vi "DAC Configure.vi"(8 "error in":errorcluster, 11 "DAC HMP4040 in":refnum<class "DAC HMP4040.lvclass">) -> (0 "error out":errorcluster, 3 "DAC HMP4040 out":refnum<class "DAC HMP4040.lvclass">)   [LabVIEW 2019, in "DAC.lvlib" / "DAC HMP4040.lvclass"]
uses:
  DAC HMP4040.lvclass
  C:/Users/krio/Documents/LV_Projects/test-stand/App/DAC/DAC.lvclass
  DAC.lvclass/DAC.ctl
  DAC HMP4040.lvclass/DAC HMP4040.ctl
  <vilib>/Instr/_visa.llb/VISA Configure Serial Port (Instr).vi
  <vilib>/Utility/error.llb/Error Cluster From Error Code.vi
  <vilib>/ErrorRing/Error Ring.xnode
  DAC.lvclass
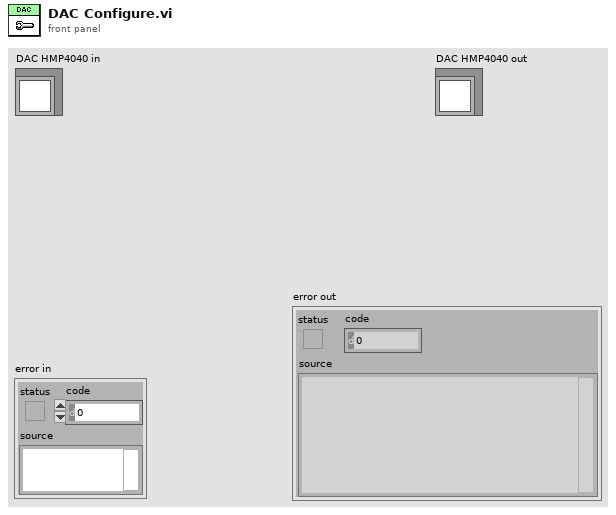
[diagram p1: front panel]
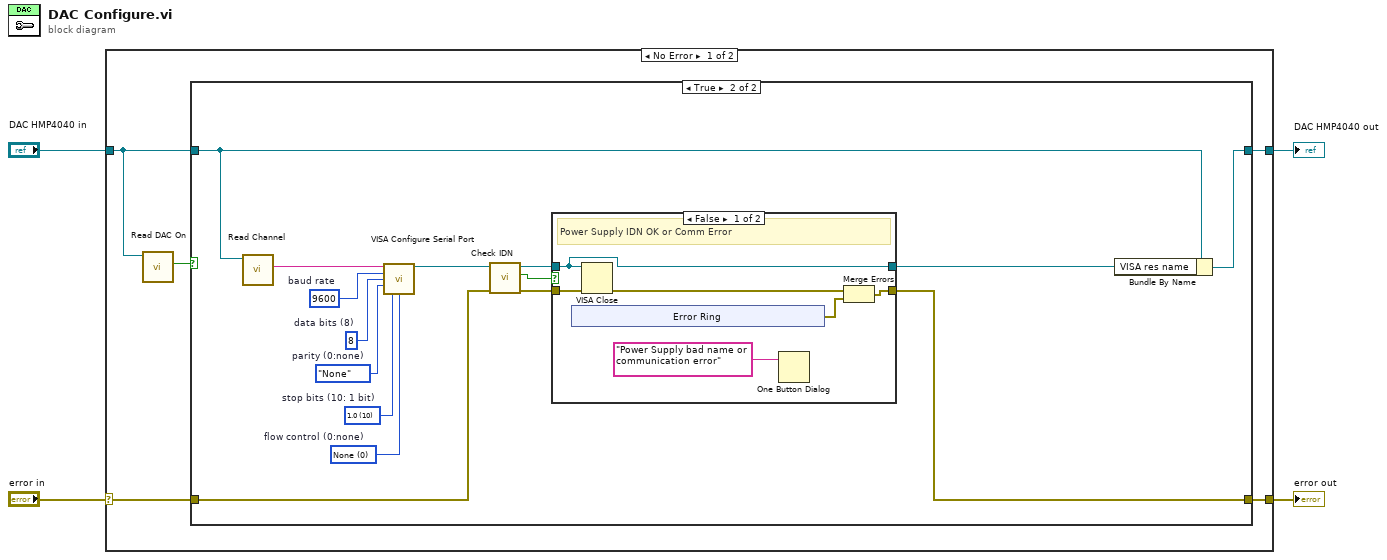
[diagram p0: block diagram]
diagram:
  n1 = case shown="No Error" "error in" {
    selector: "error in" -> [w6 w40]
    tunnel: [w5 w40] -> w4
    tunnel: [w7 w39] -> w3
    tunnel: "DAC HMP4040 in" -> [w9 w39]
    frame No Error {
      n2 = call "Read DAC On.vi"("DAC in"=w9) -> ("DAC On"=w8:bool)  [unwired: 8 in, 2 out]
      n3 = case shown="True" w8 {
        tunnel: w9 -> [w11 w21]
        tunnel: [w11 w26] -> w7
        tunnel: w6 -> [w10 w17]
        tunnel: [w10 w12] -> w5
        frame False {
        }
        frame True {
          w19 = u16 0 items=["None", "XON/XOFF", "RTS/CTS", "XON/XOFF & RTS/CTS", "DTR/DSR", "XON/XOFF & DTR/DSR"]  # flow control (0:none)
          w22 = u16 10 items=["1.0"=10, "1.5"=15, "2.0"=20]  # stop bits (10: 1 bit)
          w23 = enum16{"None", "Odd", "Even", "Mark", "Space"}."None"  # parity (0:none)
          w24 = u16 8  # data bits (8)
          w25 = u32 9600  # baud rate
          n4 = call "Read Channel.vi"("DAC in"=w21) -> ("Channel"=w20:string)  [unwired: 8 in, 2 out]
          n5 = call-poly "VISA Configure Serial Port"("VISA resource name"=w20, "baud rate (9600)"=w25, "data bits (8)"=w24, "parity (0:none)"=w23, "stop bits (10: 1 bit)"=w22, "flow control (0:none)"=w19) -> ("VISA resource name out"=w18:refnum<visa-resource-name>)  [unwired: 8 in, 1 out]
          n6 = call "Check IDN.vi"("error in"=w17, "VISA Refnum in"=w18) -> ("error out"=w13:errorcluster, "IDN OK?"=w14:bool, "VISA Refnum out"=w16:refnum<visa-resource-name>)  [unwired: 7 in]
          n7 = case shown="False" w14 {
            tunnel: w16 -> [w27 w38]
            tunnel: [w27 w38] -> w15
            tunnel: w13 -> [w30 w37]
            tunnel: [w28 w37] -> w12
            frame False {
              # "Power Supply IDN OK or Comm Error"
              n8 = xnode "Error Ring"() -> ("error out"=w31:errorcluster)
              n9 = VISA Close(VISA resource name=w27, error in (no error)=w30) -> (error out=w29:errorcluster)
              n10 = One Button Dialog(message="Power Supply bad name or communication error" ("format string")) -> ()  [unwired: 1 in, 1 out]
              n11 = Merge Errors(w29, w31) -> (w28:errorcluster)
            }
            frame True {
              # "Power Supply IDN OK"
            }
          }
          n12 = Bundle By Name(cluster=w21, "VISA res name"=w15) -> (w26:refnum<class "DAC HMP4040.lvclass">)
        }
      }
    }
    frame Error {
    }
  }
  "error out" <- w4
  "DAC HMP4040 out" <- w3
